vi "Code Report CLI.vi"(11 "Command Line Args":string[](array[string])=["SearchPath=\"..\\..\\Source\\\"", "ReportPath=\"..\\..\\CodeReport.xml\"", "Recursive=true", "ListParams=true", "ListDocs=true"]) -> (2 "Return Message":string="No Error", 3 "Return Code":i32)   [LabVIEW 2016]
uses:
  Typedefs/Command Line Arguments.ctl
  <vilib>/Utility/error.llb/DialogType.ctl
  <vilib>/ni/Simple XML/_polymorphics/Create Tag - Root.vi
  <vilib>/ni/Simple XML/_polymorphics/Create Tag - Child.vi
  <vilib>/ni/Simple XML/_polymorphics/Create Tag - Child with Text.vi
  <vilib>/xml/Close Reference(Node).vi
  <vilib>/xml/NI_XML.lvlib
  <vilib>/ni/Simple XML/Simple XML.lvlib
  <resource>/objmgr/DOMUserDefRef.rc
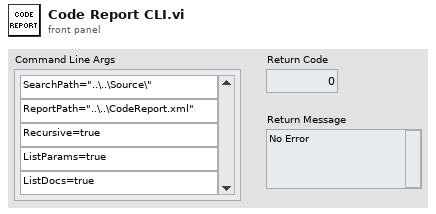
[diagram p1: front panel]
types:
  T1 = typedef "DialogType.ctl" = u16
  T2 = typedef "Command Line Arguments.ctl" = cluster{"Search Path":path, "Report Path":path, "Recursive Search?":bool, "List Parameters?":bool, "Include Documentation?":bool}
  T3 = enum32{"invalid VI type", "Standard VI", "Control VI", "Global VI", "Polymorphic VI", "Configuration VI", "SubSystem", "Facade VI", "Method VI", "Statechart Diagram VI"}
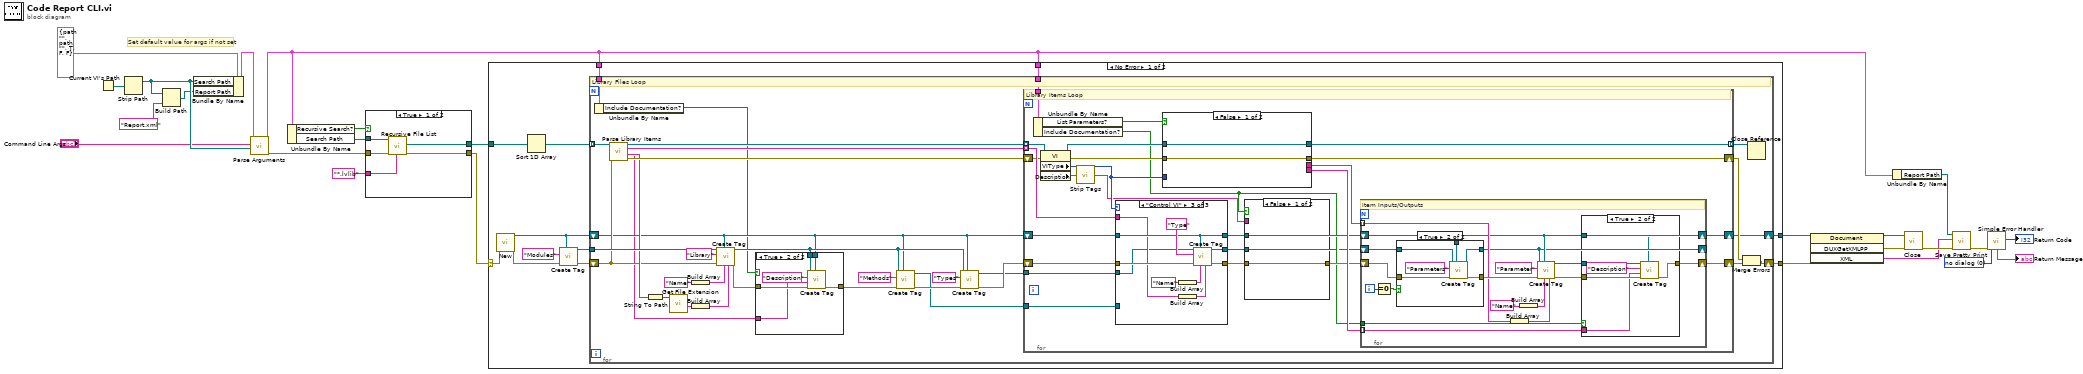
[diagram p0: block diagram]
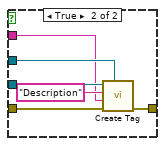
[diagram p3: hidden frame]
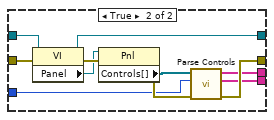
[diagram p4: hidden frame]
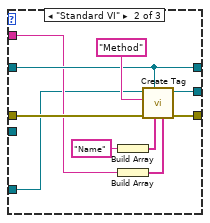
[diagram p6: hidden frame]
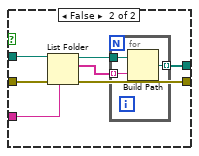
[diagram p10: hidden frame]
diagram:
  w5 = T1 0 items=["no dialog", "OK message", "continue or stop message", "OK message + warnings", "continue/stop + warnings"] ("type of dialog (OK msg:1)")
  # "Set default value for args if not set"
  n1 = Current VI's Path() -> (path=w10:path)
  n2 = Strip Path(path=w10) -> (stripped path=w19:path)  [unwired: 1 out]
  n3 = Build Path(base path=w19, name or relative path="Report.xml") -> (appended path=w7:path)
  n4 = Bundle By Name(cluster=T2 {"Search Path"=path "", "Report Path"=path "", "Recursive Search?"=TRUE, "List Parameters?"=FALSE, "Include Documentation?"=FALSE} ("Default Values"), "Search Path"=w19, "Report Path"=w7) -> (w8:T2)
  n5 = call "Parse Arguments.vi"("Working Directory"=w19, "Command Line Args"="Command Line Args", "Parameters in"=w8) -> ("error constant"=w25:errorcluster, "Parameters out"=w1:T2)  [unwired: 7 in]
  n6 = Unbundle By Name(w1) -> ("Recursive Search?"=w12:bool, "Search Path"=w16:path)
  n7 = case shown="True" w12 {
    tunnel: "*.lvlib" ("pattern") -> [w28 w35]
    tunnel: w16 -> [w27 w34]
    tunnel: w25 -> [w30 w37]
    tunnel: [w29 w36] -> w20
    tunnel: [w26 w31] -> w2
    frame True {
      n8 = call <vilib>:"Recursive File List.vi"("pattern"=w28, "error in (no error)"=w30, "Folder Path"=w27) -> ("error out"=w29:errorcluster, "All Files in Dir"=w26:path[])  [unwired: 4 in, 3 out]
    }
    frame False {
      n9 = List Folder(path=w34, pattern=w35, error in=w37) -> (path out=w33:path, filenames=w32:string[], error out=w36:errorcluster)  [unwired: 1 in, 1 out]
      n10 = for {
        tunnel: w33 -> [w40]
        tunnel: w32 -> [w39] mode=indexing
        tunnel: [w38] -> w31 mode=indexing
        n11 = Build Path(base path=w40, name or relative path=w39) -> (appended path=w38:path)
      }
    }
  }
  n12 = case shown="No Error" w20 {
    selector: w20 -> [w50 w191]
    tunnel: [w52 w191] -> w22
    tunnel: [w48 _] -> w11
    tunnel: w1 -> [w47 _]
    tunnel: w2 -> [w43 _]
    tunnel: w1 -> [w41 _]
    frame No Error {
      n13 = call <vilib>:"New.vi"("error in (no error)"=w50) -> ("error out"=w51:errorcluster, "DOM document out"=w44:refnum<k20>)  [unwired: 7 in]
      n14 = Sort 1D Array(array=w43) -> (sorted array=w42:path[])
      n15 = call-poly <vilib>:"Create Tag.vi"("DOM document reference"=w44, "error in (no error)"=w51, "Tag Name"="Modules") -> ("error out"=w49:errorcluster, "Element reference"=w45:refnum<k20>)  [unwired: 7 in]
      n16 = for {
        tunnel: w42 -> [w80] mode=indexing
        tunnel: w45 -> [w79]
        shift-right: [w71] -> w48
        shift-left: w44 -> [w58]
        shift-right: [w82] -> w52
        shift-left: w49 -> [w60]
        tunnel: w47 -> [w70]
        tunnel: w41 -> [w54]
        # "Library Files Loop"
        n17 = Unbundle By Name(w54) -> ("Include Documentation?"=w53:bool)
        n18 = call "Parse Library Items.vi"("Library Path"=w80, "error in (no error)"=w60) -> ("References"=w62:refnum<vi>[], "File Names"=w61:string[], "Display Name"=w63:string, "Description"=w55:string, "error out"=w83:errorcluster)  [unwired: 9 in]
        n19 = String To Path(string=w63) -> (path=w74:path)
        n20 = call <vilib>:"Get File Extension.vi"("file"=w74) -> ("filename without extension"=w73:string)  [unwired: 6 in, 4 out]
        n21 = Build Array("Name" ("Tag Name")) -> (w75:string[])
        n22 = Build Array(w73) -> (w77:string[])
        n23 = call-poly <vilib>:"Create Tag.vi"("Attr Values"=w77, "Attr Names"=w75, "DOM Document reference"=w58, "error in (no error)"=w60, "Tag Name"="Library", "Parent Element reference"=w79) -> ("error out"=w57:errorcluster, "Child Element reference"=w59:refnum<k20>)  [unwired: 4 in]
        n24 = case shown="True" w53 {
          tunnel: w59 -> [_ w90]
          tunnel: w58 -> [_ w89]
          tunnel: w57 -> [w85 w88]
          tunnel: [w85 w87] -> w56
          tunnel: w55 -> [_ w86]
          frame False {
          }
          frame True {
            n25 = call-poly <vilib>:"Create Tag.vi"("DOM document reference"=w89, "error in (no error)"=w88, "Text Data"=w86, "Tag Name"="Description", "Parent Element reference"=w90) -> ("error out"=w87:errorcluster)  [unwired: 5 in, 1 out]
          }
        }
        n26 = call-poly <vilib>:"Create Tag.vi"("DOM Document reference"=w58, "error in (no error)"=w56, "Tag Name"="Methods", "Parent Element reference"=w59) -> ("error out"=w69:errorcluster, "Child Element reference"=w65:refnum<k20>)  [unwired: 6 in]
        n27 = call-poly <vilib>:"Create Tag.vi"("DOM Document reference"=w58, "error in (no error)"=w69, "Tag Name"="Types", "Parent Element reference"=w59) -> ("error out"=w68:errorcluster, "Child Element reference"=w64:refnum<k20>)  [unwired: 6 in]
        n28 = for {
          tunnel: [w101] -> w72 mode=indexing
          shift-right: [w110] -> w71
          shift-left: w58 -> [w112]
          shift-right: [w114] -> w84
          shift-left: w68 -> [w116]
          shift-right: [w113] -> w81
          shift-left: w83 -> [w102]
          tunnel: w70 -> [w109]
          tunnel: w65 -> [w105]
          tunnel: w64 -> [w104]
          tunnel: w62 -> [w99] mode=indexing
          tunnel: w61 -> [w103] mode=indexing
          # "Library Items Loop"
          n29 = Unbundle By Name(w109) -> ("List Parameters?"=w108:bool, "Include Documentation?"=w95:bool)
          n30 = property class="VI"(reference=w99, error in=w102) -> (reference out=w98:refnum<vi>, error out=w100:errorcluster, "VIType"=w107:T3, "Description"=w94:string)
          n31 = call "Strip Tags.vi"("Description in"=w94) -> ("Description out"=w92:string)  [unwired: 14 in]
          n32 = case shown="\"Control VI\"" w107 {
            tunnel: w116 -> [w138 w148 w158]
            tunnel: w103 -> [_ w141 w151]
            tunnel: [w138 w147 w157] -> w115
            tunnel: w112 -> [w137 w145 w155]
            tunnel: [w137 w145 w155] -> w96
            tunnel: [_ w144 w154] -> w93
            tunnel: w105 -> [_ w140 _]
            tunnel: w104 -> [_ _ w150]
            frame Default {
            }
            frame "Standard VI" {
              n33 = Build Array("Name" ("Tag Name")) -> (w142:string[])
              n34 = Build Array(w141) -> (w139:string[])
              n35 = call-poly <vilib>:"Create Tag.vi"("Attr Values"=w139, "Attr Names"=w142, "DOM Document reference"=w145, "error in (no error)"=w148, "Tag Name"="Method", "Parent Element reference"=w140) -> ("error out"=w147:errorcluster, "Child Element reference"=w144:refnum<k20>)  [unwired: 4 in]
            }
            frame "Control VI" {
              n36 = Build Array("Name" ("Tag Name")) -> (w152:string[])
              n37 = Build Array(w151) -> (w149:string[])
              n38 = call-poly <vilib>:"Create Tag.vi"("Attr Values"=w149, "Attr Names"=w152, "DOM Document reference"=w155, "error in (no error)"=w158, "Tag Name"="Type", "Parent Element reference"=w150) -> ("error out"=w157:errorcluster, "Child Element reference"=w154:refnum<k20>)  [unwired: 4 in]
            }
          }
          n39 = case shown="False" w108 {
            tunnel: [_ w134] -> w111
            tunnel: [w125 w135] -> w113
            tunnel: w107 -> [_ w131]
            tunnel: [_ w133] -> w106
            tunnel: [w124 w128] -> w101
            tunnel: w98 -> [w124 w129]
            tunnel: w100 -> [w125 w130]
            frame False {
            }
            frame True {
              n40 = property class="VI"(reference=w129, error in=w130) -> (reference out=w128:refnum<vi>, error out=w127:errorcluster, "Panel"=w126:refnum<vi>)
              n41 = property class="Pnl"(reference=w126, error in=w127) -> (error out=w136:errorcluster, "Controls[]"=w132:refnum<vi>[])  [unwired: 1 out]
              n42 = call "Parse Controls.vi"("error in (no error)"=w136, "VI Type"=w131, "Controls[]"=w132) -> ("error out"=w135:errorcluster, "Control Descriptions"=w133:string[], "Control Names"=w134:string[])  [unwired: 5 in, 1 out]
            }
          }
          n43 = case shown="False" w95 {
            tunnel: w115 -> [w117 w123]
            tunnel: [w117 w122] -> w97
            tunnel: w93 -> [_ w121]
            tunnel: w96 -> [_ w120]
            tunnel: w92 -> [_ w118]
            frame False {
            }
            frame True {
              n44 = call-poly <vilib>:"Create Tag.vi"("DOM document reference"=w120, "error in (no error)"=w123, "Text Data"=w118, "Tag Name"="Description", "Parent Element reference"=w121) -> ("error out"=w122:errorcluster)  [unwired: 5 in, 1 out]
            }
          }
          n45 = for {
            shift-right: [w167] -> w114
            shift-left: w97 -> [w175]
            tunnel: w111 -> [w168] mode=indexing
            shift-right: [w165] -> w110
            shift-left: w96 -> [w165]
            tunnel: w106 -> [w164] mode=indexing
            tunnel: w95 -> [w163]
            shift-right: [w161] -> _
            shift-left: w93 -> [w162]
            i -> [w160]
            # "Item Inputs/Outputs"
            n46 = Equal To 0?(x=w160) -> (x = 0?=w159:bool)
            n47 = case shown="True" w159 {
              tunnel: w175 -> [w176 w183]
              tunnel: [w176 w182] -> w173
              tunnel: w165 -> [_ w180]
              tunnel: w162 -> [w177 w179]
              tunnel: [w177 w178] -> w161
              frame False {
              }
              frame True {
                n48 = call-poly <vilib>:"Create Tag.vi"("DOM Document reference"=w180, "error in (no error)"=w183, "Tag Name"="Parameters", "Parent Element reference"=w179) -> ("error out"=w182:errorcluster, "Child Element reference"=w178:refnum<k20>)  [unwired: 6 in]
              }
            }
            n49 = Build Array(w168) -> (w169:string[])
            n50 = Build Array("Name" ("Tag Name")) -> (w170:string[])
            n51 = call-poly <vilib>:"Create Tag.vi"("Attr Values"=w169, "Attr Names"=w170, "DOM Document reference"=w165, "error in (no error)"=w173, "Tag Name"="Parameter", "Parent Element reference"=w161) -> ("error out"=w174:errorcluster, "Child Element reference"=w166:refnum<k20>)  [unwired: 4 in]
            n52 = case shown="True" w163 {
              tunnel: w174 -> [w184 w190]
              tunnel: [w184 w189] -> w167
              tunnel: w166 -> [_ w188]
              tunnel: w165 -> [_ w186]
              tunnel: w164 -> [_ w185]
              frame False {
              }
              frame True {
                n53 = call-poly <vilib>:"Create Tag.vi"("DOM document reference"=w186, "error in (no error)"=w190, "Text Data"=w185, "Tag Name"="Description", "Parent Element reference"=w188) -> ("error out"=w189:errorcluster)  [unwired: 5 in, 1 out]
              }
            }
          }
        }
        n54 = Merge Errors(w81, w84) -> (w82:errorcluster)
        n55 = Close Reference(reference=w72) -> ()  [unwired: 1 in, 1 out]
      }
    }
    frame Error {
    }
  }
  n56 = invoke class="Document" method="DUXGetXMLPP"(reference=w11, error in=w22) -> (reference out=w15:refnum<k20>, error out=w23:errorcluster, "XML"=w14:string)  [unwired: 2 in, 1 out]
  n57 = Unbundle By Name(w1) -> ("Report Path"=w13:path)
  n58 = call-poly <vilib>:"Close.vi"("error in (no error)"=w23, "node"=w15) -> ("error out"=w24:errorcluster)  [unwired: 7 in]
  n59 = call <vilib>:"Save Pretty Print.vi"("error in (no error)"=w24, "Pretty XML String"=w14, "XML file path"=w13) -> ("error out"=w21:errorcluster)  [unwired: 7 in, 1 out]
  n60 = call <vilib>:"Simple Error Handler.vi"("type of dialog (OK msg:1)"=w5, "error in (no error)"=w21) -> ("code out"=→"Return Code":i32, "message"=→"Return Message":string)  [unwired: 3 in, 3 out]
